vi "VIH Project - Verify CSS,JS,Template Files - File  Rule.vi"(10 "File Rule":T1, 11 "File path":path) -> (2 "Bad files":path[](array[path]))   [LabVIEW 2014]
doc: "::: VI Helpeks :::\nCopyright (c) 2000-2026 Konstantin Shifershteyn. All rights reserved."
uses:
  _VIH HelpGen.llb/VIH HelpGen Typedef - Cluster - File Rule.ctl
  _VIH HelpGen.llb/VIH HelpGen Typedef - Enum - Default,Enable,Disable.ctl
  _VIH HelpGen.llb/VIH HelpGen Typedef - Cluster - File Rule - Source Paths.ctl
  _VIH HelpGen.llb/VIH HelpGen Typedef - Cluster - File Rule - Target Paths.ctl
  _VIH HelpGen.llb/VIH HelpGen Typedef - Enum - Description Mode.ctl
  _VIH HelpGen.llb/VIH HelpGen Typedef - Cluster - Control Rule.ctl
  _VIH HelpGen.llb/VIH HelpGen Typedef - Cluster - Enum Value Info.ctl
  _VIH HelpGen.llb/VIH HelpGen Typedef - Cluster - Group Rule - Flags.ctl
panel:
  # "VI Helpeks\nCopyright (c) 2012-2026 Konstantin Shifershteyn"
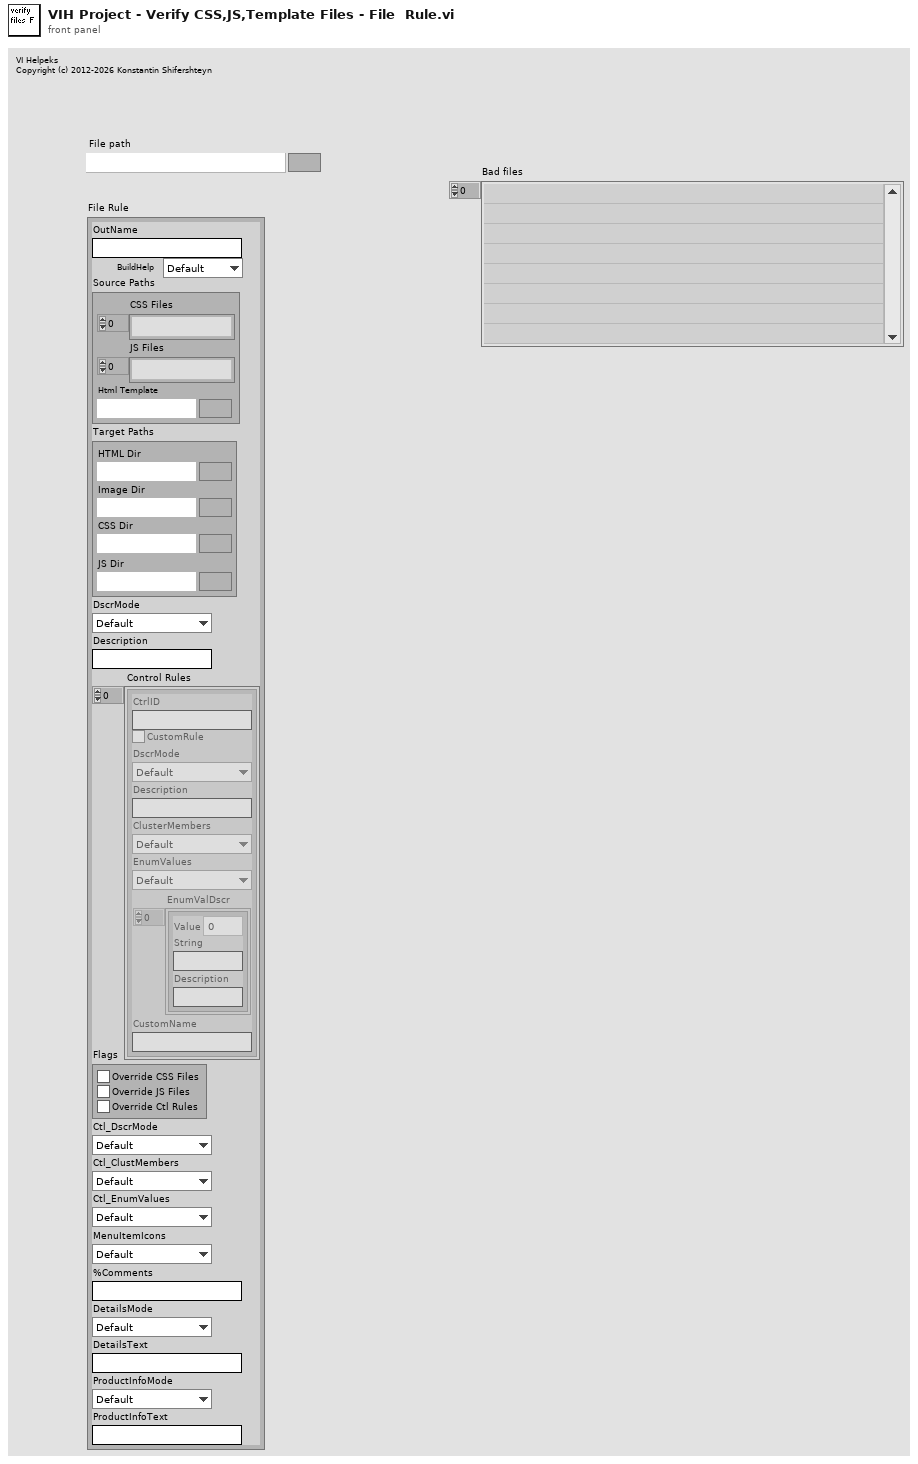
[diagram p1: front panel]
types:
  T1 = typedef "VIH HelpGen Typedef - Cluster - File Rule.ctl" = cluster{"OutName":string, "BuildHelp":T2, "Source Paths":T3, "Target Paths":T4, "DscrMode":T5, "Description":string, "Control Rules":T6[], "Flags":T8, "Ctl_DscrMode":T5, "Ctl_ClustMembers":T2, "Ctl_EnumValues":T2, "MenuItemIcons":T2, "%Comments":string, "DetailsMode":T5, "DetailsText":string, "ProductInfoMode":T2, "ProductInfoText":string}
  T2 = typedef "VIH HelpGen Typedef - Enum - Default,Enable,Disable.ctl" = enum16{"Default", "Enable", "Disable"}
  T3 = typedef "VIH HelpGen Typedef - Cluster - File Rule - Source Paths.ctl" = cluster{"CSS Files":path[], "JS Files":path[], "Html Template":path}
  T4 = typedef "VIH HelpGen Typedef - Cluster - File Rule - Target Paths.ctl" = cluster{"HTML Dir":path, "Image Dir":path, "CSS Dir":path, "JS Dir":path}
  T5 = typedef "VIH HelpGen Typedef - Enum - Description Mode.ctl" = enum16{"Default", "Description", "Description1", "Description2", "Custom", "None"}
  T6 = typedef "VIH HelpGen Typedef - Cluster - Control Rule.ctl" = cluster{"CtrlID":string, "CustomRule":bool, "DscrMode":T5, "Description":string, "ClusterMembers":T2, "EnumValues":T2, "EnumValDscr":T7[], "CustomName":string}
  T7 = typedef "VIH HelpGen Typedef - Cluster - Enum Value Info.ctl" = cluster{"Value":ext, "String":string, "Description":string}
  T8 = typedef "VIH HelpGen Typedef - Cluster - Group Rule - Flags.ctl" = cluster{"Override CSS Files":bool, "Override JS Files":bool, "Override Ctl Rules":bool}
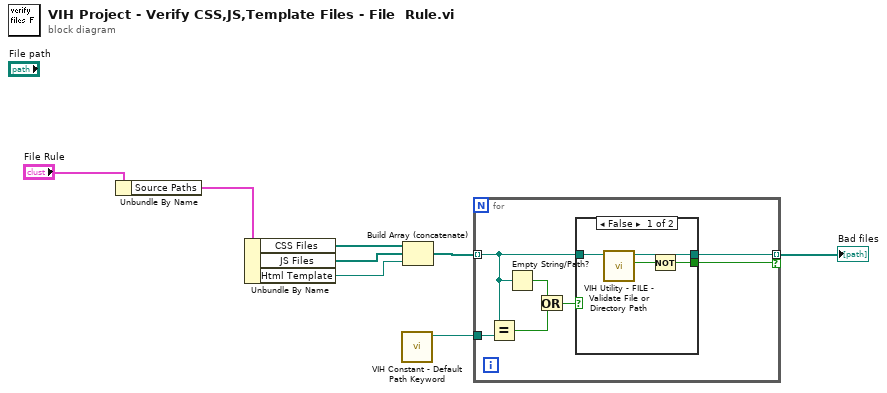
[diagram p0: block diagram]
diagram:
  n1 = Unbundle By Name("File Rule") -> ("Source Paths"=w7:T3)
  n2 = Unbundle By Name(w7) -> ("CSS Files"=w6:path[], "JS Files"=w5:path[], "Html Template"=w4:path)
  n3 = call "VIH Constant - Default Path Keyword.vi"() -> ("<default> path"=w2:path)  [unwired: 11 in]
  n4 = Build Array (concatenate)(w6, w5, w4) -> (w3:path[])
  n5 = for {
    tunnel: w3 -> [w12] mode=indexing
    tunnel: w2 -> [w15]
    tunnel: [w11] -> w1 mode=indexing if=w9
    n6 = Equal?(x=w12, y=w15) -> (x = y?=w13:bool)
    n7 = Empty String/Path?(string/path=w12) -> (empty?=w14:bool)
    n8 = Or(x=w14, y=w13) -> (x .or. y?=w10:bool)
    n9 = case shown="False" w10 {
      tunnel: w12 -> [w19 w20]
      tunnel: [w18 w20] -> w11
      tunnel: [w16 _] -> w9
      frame False {
        n10 = call "VIH Utility - FILE - Validate File or Directory Path.vi"("Path"=w19) -> ("file"=w17:bool, "dup Path"=w18:path)  [unwired: 6 in, 3 out]
        n11 = Not(x=w17) -> (.not. x?=w16:bool)
      }
      frame True {
      }
    }
  }
  "Bad files" <- w1
